vi "VIPM Post Install Process.vi"(7 "vi.lib relative path (Viviota\\shared)":path=path "Viviota/shared", 8 "Error In":errorcluster, 10 "Files Installed":path[](array[path]), 11 "Package Name":string) -> (0 "Error Out":errorcluster, 2 "Files Replaced":path[](array[path]), 3 "New Files Added":path[](array[path]))   [LabVIEW 2020]
uses:
  <vilib>/Utility/file.llb/Write Delimited Spreadsheet (string).vi
  <vilib>/zip/NI_Unzip.lvlib
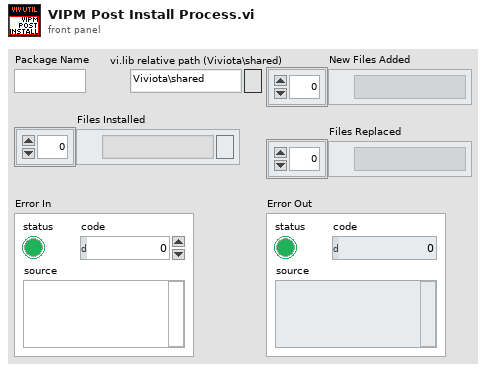
[diagram p1: front panel]
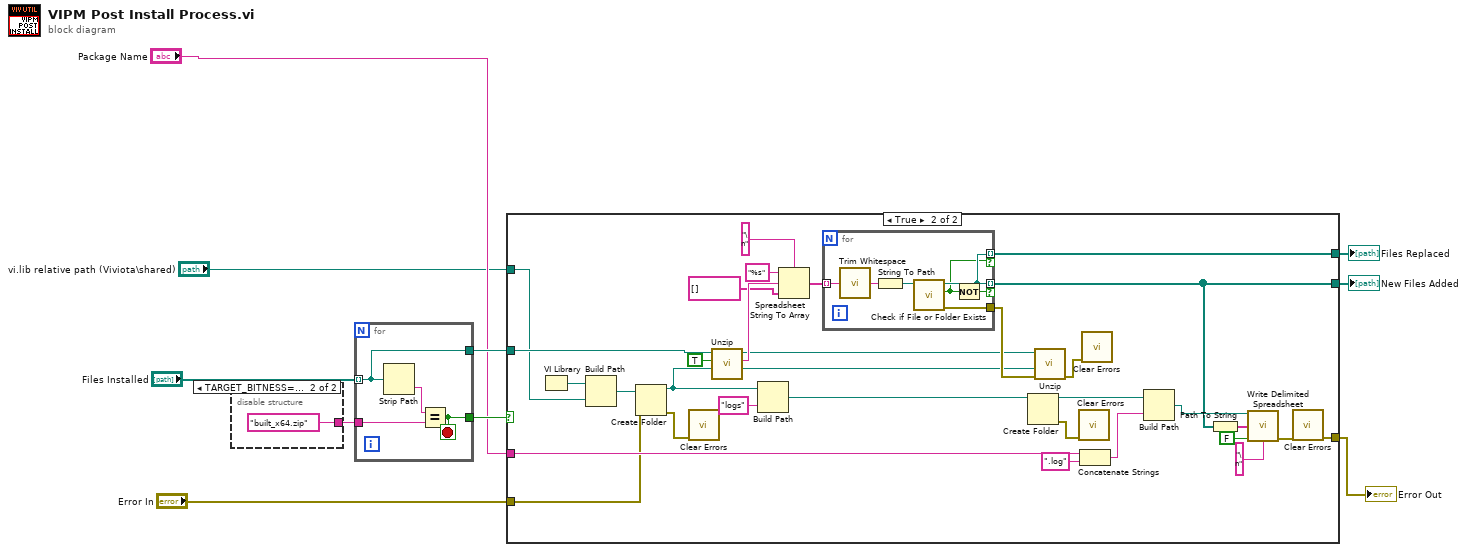
[diagram p0: block diagram]
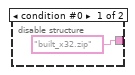
[diagram p2: hidden frame]
diagram:
  n1 = disable-structure shown="TARGET_BITNESS==64" {
    disable-tunnel: ["built_x32.zip" "built_x64.zip"] -> w8
    frame condition #0 {
    }
    frame condition #1 (active) {
    }
  }
  n2 = for {
    tunnel: w8 -> [w15]
    tunnel: "Files Installed" -> [w13] mode=indexing
    tunnel: [w14] -> w9
    tunnel: [w13] -> w10
    stop <- w14 stop-if-true
    n3 = Strip Path(path=w13) -> (name=w16:string)  [unwired: 1 out]
    n4 = Equal?(x=w16, y=w15) -> (x = y?=w14:bool)
  }
  n5 = case shown="True" w9 {
    tunnel: w10 -> [_ w24]
    tunnel: "Package Name" -> [_ w40]
    tunnel: [_ w22] -> w2
    tunnel: [_ w21] -> w5
    tunnel: [_ w20] -> w4
    tunnel: "Error In" -> [_ w18]
    tunnel: "vi.lib relative path (Viviota\\shared)" -> [_ w17]
    frame False {
    }
    frame True {
      n6 = VI Library() -> (path=w46:path)
      n7 = Build Path(base path=w46, name or relative path=w17) -> (appended path=w45:path)
      n8 = Create Folder(path (use dialog)=w45, error in=w18) -> (created path=w23:path, error out=w44:errorcluster)  [unwired: 1 in, 1 out]
      n9 = call <vilib>:"Clear Errors.vi"("error in (no error)"=w44) -> ()  [unwired: 5 in, 2 out]
      n10 = call <vilib>:"Unzip.vi"("Target directory (same as Zip file if empty)"=w23, "Preview only?"=TRUE, "Zip file"=w24) -> ("Preview"=w30:string)  [unwired: 6 in, 2 out]
      n11 = Build Path(base path=w23, name or relative path="logs") -> (appended path=w42:path)
      n12 = Spreadsheet String To Array(delimiter (Tab)="\n", format string="%s", spreadsheet string=w30, array type (2D Dbl)=string[] []) -> (array=w26:string[])
      n13 = for {
        tunnel: w26 -> [w53] mode=indexing
        tunnel: [w49] -> w21 mode=indexing if=w51
        tunnel: [w50] -> w25
        tunnel: [w49] -> w20 mode=indexing if=w48
        n14 = call <vilib>:"Trim Whitespace.vi"("string"=w53) -> ("trimmed string"=w47:string)  [unwired: 1 in]
        n15 = String To Path(string=w47) -> (path=w52:path)
        n16 = call <vilib>:"Check if File or Folder Exists.vi"("path"=w52) -> ("error out"=w50:errorcluster, "file or folder exists?"=w48:bool, "dup path"=w49:path)  [unwired: 8 in]
        n17 = Not(x=w48) -> (.not. x?=w51:bool)
      }
      n18 = Create Folder(path (use dialog)=w42) -> (created path=w37:path, error out=w41:errorcluster)  [unwired: 2 in, 1 out]
      n19 = call <vilib>:"Unzip.vi"("error in (no error)"=w25, "Target directory (same as Zip file if empty)"=w23, "Zip file"=w24) -> ("error out"=w19:errorcluster)  [unwired: 6 in, 2 out]
      n20 = call <vilib>:"Clear Errors.vi"("error in (no error)"=w41) -> ()  [unwired: 5 in, 2 out]
      n21 = Concatenate Strings(w40, ".log" ("string")) -> (w36:string)
      n22 = call <vilib>:"Clear Errors.vi"("error in (no error)"=w19) -> ()  [unwired: 5 in, 2 out]
      n23 = Build Path(base path=w37, name or relative path=w36) -> (appended path=w35:path)
      n24 = Path To String(path=w21) -> (string=w38:string[])
      n25 = call-poly <vilib>:"Write Delimited Spreadsheet.vi"("file path (dialog if empty)"=w35, "1D data"=w38, "append to file? (new file:F)"=FALSE, "delimiter (\\t)"="\n" ("delimiter (\\t)")) -> ("error out"=w33:errorcluster)  [unwired: 10 in, 1 out]
      n26 = call <vilib>:"Clear Errors.vi"("error in (no error)"=w33) -> ("error out"=w22:errorcluster)  [unwired: 5 in, 1 out]
    }
  }
  "New Files Added" <- w5
  "Files Replaced" <- w4
  "Error Out" <- w2
